vi "lvmcp_constrep.vi"() -> ()   [LabVIEW 2015]
panel:
  out "error out":errorcluster
  in  "representation":u16
  in  "reference":refnum<vi>
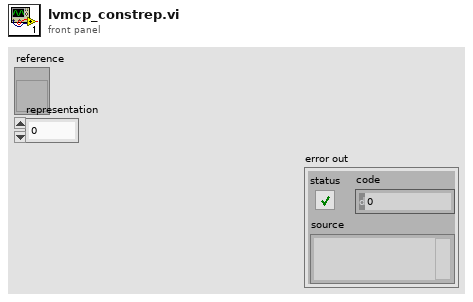
[diagram p1: front panel]
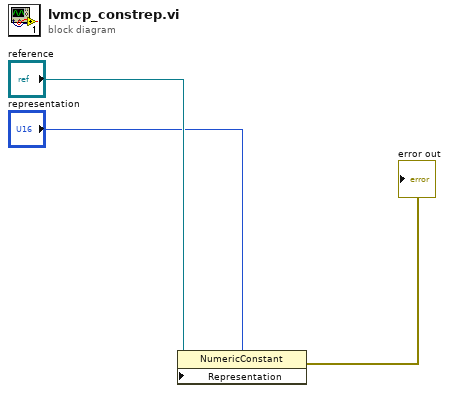
[diagram p0: block diagram]
diagram:
  n1 = property class="NumericConstant"(reference="reference", "Representation"="representation") -> (error out=→"error out":errorcluster)  [unwired: 1 in, 1 out]
